vi "Build Error Response.vi"(8 "error in":errorcluster, 11 "error json":string) -> (0 "error out":errorcluster, 3 "response":string)   [LabVIEW 2020, in "MCP Server.lvlib"]
doc: "Turns a LabVIEW error that a request handler left on the error wire into a JSON-RPC error response, so that no flattened error cluster, VI call chain or markup leaves the server.\n\nerror json is the error cluster flattened to JSON (status, code, source), as Flatten To JSON produces it.\n\nJSON-RPC code: -32602 (invalid params) for LabVIEW error 131214 (unknown prompt) and 402841 (JSON item not found, for example missing arguments), -32002 (resource not found) for 131216, -32603 (internal error) for everything else.\nThe message is cleaned by Clean Error Message.vi.\n\nThe response carries id 0. Restore Request ID.vi puts the id of the request in afterwards."
uses:
  MCP Server.lvlib
  d871bd14-a450-4504-a281-86be7a79edce.vi
  <vilib>/JDP Science/JSONtext/Next JSON Value.vi
  <vilib>/JDP Science/JSONtext/String Subset.vi
  <vilib>/JDP Science/JSONtext/Parsing/Advance past next JSON Value (inlined COPY).vi
  <vilib>/JDP Science/JSONtext/Parsing/Advance past whitespace.vi
  <vilib>/JDP Science/JSONtext/Parsing/Advance past String.vi
  <vilib>/JDP Science/JSONtext/Parsing/Advance past Number.vi
  <vilib>/JDP Science/JSONtext/Parsing/Advance past Line Ending.vi
  <vilib>/JDP Science/JSONtext/Parsing/Parse Full Path or Item Name.vi
  <vilib>/JDP Science/JSONtext/Parsing/Advance past Array.vi
  <vilib>/JDP Science/JSONtext/Parsing/Advance past Object.vi
  <vilib>/JDP Science/JSONtext/support/Error Cluster From Code.vi
  <vilib>/JDP Science/JSONtext/Offset/Find Item Locations by Path.vi
  <vilib>/JDP Science/JSONtext/JSON text to Variant.vi
  <vilib>/JDP Science/JSONtext/LVClass Serializer/JSONtext LVClass Serializer.lvclass
  <vilib>/JDP Science/JSONtext/JSONtext.lvlib
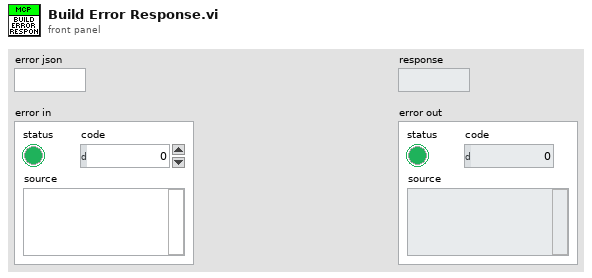
[diagram p1: front panel]
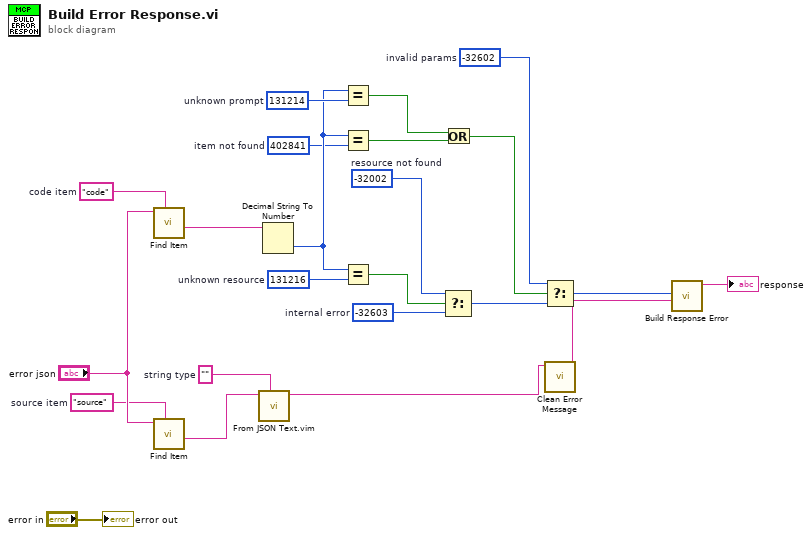
[diagram p0: block diagram]
diagram:
  w7 = -32602  # invalid params
  w10 = -32002  # resource not found
  w8 = -32603  # internal error
  w13 = 402841  # item not found
  w15 = 131216  # unknown resource
  w16 = 131214  # unknown prompt
  w18 = ""  # string type
  w20 = "source"  # source item
  w23 = "code"  # code item
  n1 = call <vilib>:"Find Item.vi"("$Path or Item Name"=w23, "JSON"="error json") -> ("<JSON>"=w22:string)  [unwired: 6 in, 3 out]
  n2 = call <vilib>:"Find Item.vi"("$Path or Item Name"=w20, "JSON"="error json") -> ("<JSON>"=w19:string)  [unwired: 6 in, 3 out]
  n3 = call "From JSON Text.vim"("Data Type and Default Value"=w18, "JSON"=w19) -> ("Data out"=w17:string)  [unwired: 8 in, 1 out]
  n4 = Decimal String To Number(string=w22) -> (number=w14:i32)  [unwired: 2 in, 1 out]
  n5 = Equal?(x=w14, y=w16) -> (x = y?=w12:bool)
  n6 = Equal?(x=w14, y=w13) -> (x = y?=w11:bool)
  n7 = Equal?(x=w14, y=w15) -> (x = y?=w9:bool)
  n8 = Select(t=w10, s=w9, f=w8) -> (s? t:f=w5:i32)
  n9 = Or(x=w12, y=w11) -> (x .or. y?=w6:bool)
  n10 = Select(t=w7, s=w6, f=w5) -> (s? t:f=w4:i32)
  n11 = call "Clean Error Message.vi"("source"=w17) -> ("message"=w1:string)  [unwired: 10 in]
  n12 = call "Build Response Error.vi"("message"=w1, "code"=w4) -> ("MCP message out"=→"response":string)  [unwired: 8 in, 1 out]
  "error out" <- "error in"
